vi "Parse Search Fundamental Frequency.vi"(8 "error in (no error)":errorcluster caption="에러 입력(에러 없음)", 10 "문자열":string, 11 "Instrument Manager 입력":refnum<class "Instrument Manager.lvclass">) -> (0 "error out":errorcluster caption="에러 출력", 1 "Center Frequency":dbl, 2 "Search Fundamental Frequency Param":T1, 3 "Instrument Manager 출력":refnum<class "Instrument Manager.lvclass">)   [LabVIEW 2023, in "Instrument Manager.lvclass"]
uses:
  Instrument Manager.lvclass
  Instrument Manager.lvclass/Instrument Manager.ctl
  Param Definition/Search Fundamental Frequency Param.ctl
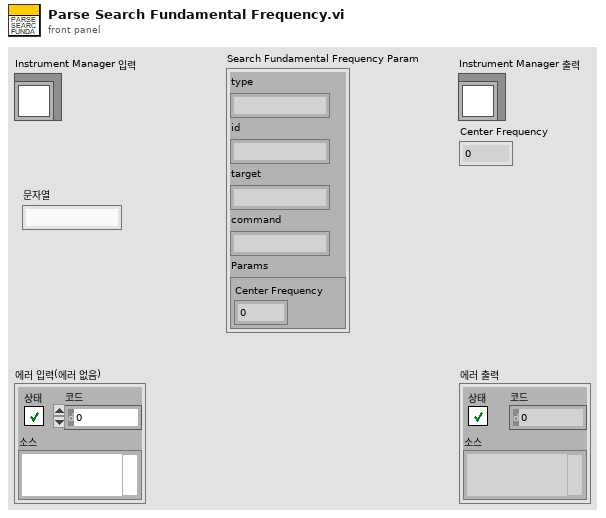
[diagram p1: front panel]
types:
  T1 = typedef "Instrument Manager.lvclass/Search Fundamental Frequency Param.ctl" = cluster{"type":string, "id":string, "target":string, "command":string, "Params":cluster{"Center Frequency":dbl}}
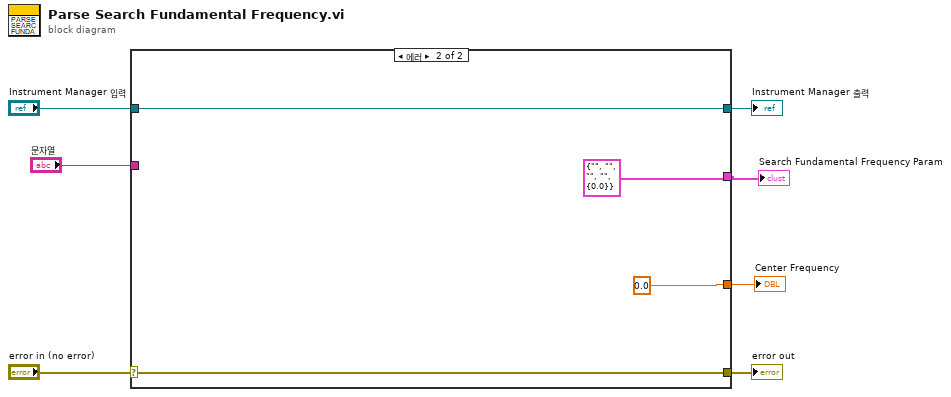
[diagram p0: block diagram]
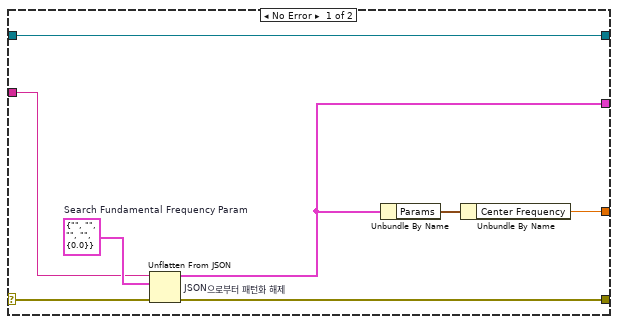
[diagram p2: hidden frame]
diagram:
  n1 = case shown="에러" "error in (no error)" {
    selector: "error in (no error)" -> [w14 w19]
    tunnel: [w8 w19] -> w6
    tunnel: [w15 w18] -> w4
    tunnel: "Instrument Manager 입력" -> [w15 w18]
    tunnel: "문자열" -> [w12 _]
    tunnel: [w10 T1 {"type"="", "id"="", "target"="", "command"="", "Params"={"Center Frequency"=0.0}} ("Search Fundamental Frequency Param")] -> w2
    tunnel: [w9 0.0 ("Center Frequency")] -> w1
    frame No Error {
      w13 = T1 {"type"="", "id"="", "target"="", "command"="", "Params"={"Center Frequency"=0.0}}  # Search Fundamental Frequency Param
      n2 = Unflatten From JSON "JSON으로부터 패턴화 해제"(JSON string=w12, type and defaults=w13, error in (no error)=w14) -> (value=w10:T1, error out=w8:errorcluster)  [unwired: 4 in]
      n3 = Unbundle By Name(w10) -> ("Params"=w11:cluster{"Center Frequency":dbl})
      n4 = Unbundle By Name(w11) -> ("Center Frequency"=w9:dbl)
    }
    frame Error {
    }
  }
  "error out" <- w6
  "Instrument Manager 출력" <- w4
  "Search Fundamental Frequency Param" <- w2
  "Center Frequency" <- w1
